vi "Update Value.vi"(6 "Time":dbl, 8 "error in (no error)":errorcluster, 11 "LoggingControl in":refnum<class "GroupLoggingControl.lvclass">) -> (0 "error out":errorcluster, 1 "Update":bool, 2 "Value":variant, 3 "LoggingControl out":refnum<class "GroupLoggingControl.lvclass">)   [LabVIEW 2020, in "VolatusGUIElements.lvlib" / "GroupLoggingControl.lvclass"]
uses:
  GroupLoggingControl.lvclass
  GroupLoggingControl.lvclass/GroupLoggingControl.ctl
  Loop Async.vi
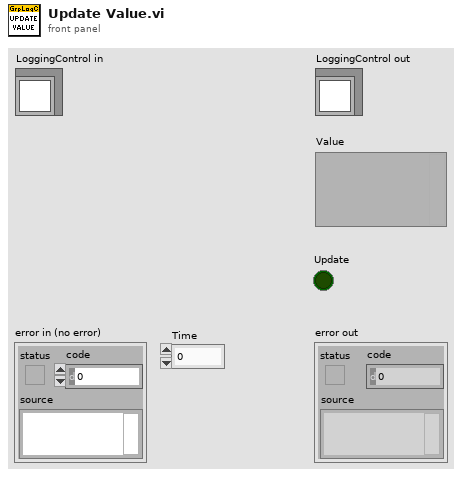
[diagram p1: front panel]
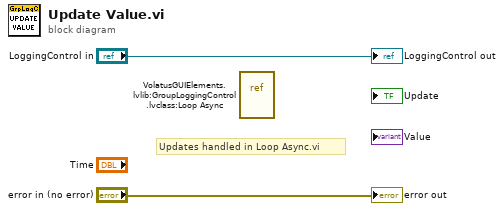
[diagram p0: block diagram]
diagram:
  # "Updates handled in Loop Async.vi"
  n1 = vi-ref "VolatusGUIElements.lvlib:GroupLoggingControl.lvclass:Loop Async.vi"() -> ()  [unwired: 1 out]
  "error out" <- "error in (no error)"
  "LoggingControl out" <- "LoggingControl in"
